vi "New UTF-8 String.vi"(7 "Input Encoding (ANSI)":T1, 9 "error in":errorcluster, 10 "String":string) -> (1 "error out":errorcluster, 2 "UTF-8 String":refnum<class "UTF-8 String.lvclass">)   [LabVIEW 2020, in "G-Unicode.lvlib" / "UTF-8 String.lvclass"]
doc: "Initializes a new UTF-8 string. <b>String</b> can be ANSI, UTF-8, or UTF-16LE encoded. The string encoding is determined automatically when <b>Encoding</b> is set to Unknown, or explicitly when set to ANSI, UTF-8, UTF-16LE or UTF-16BE.\n\nNote that automatic encoding detection isn't 100% accurate, and it is recommended to set the encoding explicitly if it is known.\n\n<b>ANSI</b> will be encoded as UTF-8 using the local codepage.\n<b>UTF-8</b> will be unchanged.\n<b>UTF-16LE</b> and <b>UTF-16BE</b> will be converted to UTF-8."
uses:
  UTF-8 String.lvclass
  Unicode/Controls/String Encoding.ctl
  UTF-8 String.lvclass/UTF-8 String.ctl
  Private/Conversion/Text to UTF-8.vi
  Private/Conversion/Polymorphic VIs/Text to UTF-8 (LabVIEW String).vi
  Private/Conversion/Encoded UTF-8 String to Encoded UTF-16LE String.vi
  Unicode/SubVIs/UTF-16 Byte Swap.vi
  Private/Conversion/UTF-8 to Text.vi
  Private/Conversion/Polymorphic VIs/UTF-8 to Text (LabVIEW String).vi
  Private/Conversion/Encoded UTF-16LE String to Encoded UTF-8 String.vi
  Unicode/Prepend BOM.vi
  Unicode/SubVIs/Byte Order Marks.vi
  Unicode/Detect BOM.vi
  Unicode/Detect String Encoding.vi
  G-Unicode.lvlib
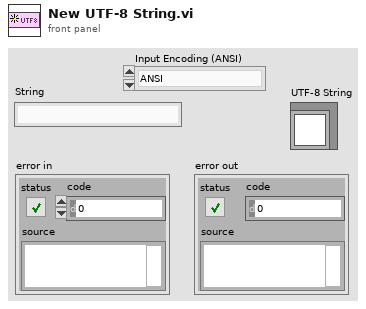
[diagram p1: front panel]
types:
  T1 = typedef "G-Unicode.lvlib/String Encoding.ctl" = enum16{"ANSI", "UTF-8", "UTF-16LE", "UTF-16BE", "Unknown"}
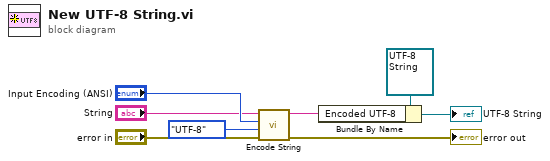
[diagram p0: block diagram]
diagram:
  n1 = call "Encode String.vi"("error in"="error in", "Output Encoding (UTF-16LE)"=String_Encoding."UTF-8", "Input Encoding (ANSI)"="Input Encoding (ANSI)", "String in"="String") -> ("error out"=→"error out":errorcluster, "String out"=w3:string)  [unwired: 6 in]
  n2 = Bundle By Name(cluster=refnum<class "UTF-8 String.lvclass"> refnum ("G-Unicode.lvlib:UTF-8.lvclass"), "Encoded UTF-8"=w3) -> (→"UTF-8 String":refnum<class "UTF-8 String.lvclass">)
